vi "RemoteVI Encode Rect PNG.vi"(8 "error in":errorcluster, 9 "compression":i32=1, 10 "rect":cluster{"x":i32, "y":i32, "w":i32, "h":i32}, 11 "pixmap":u32[][](array[numeric])) -> (0 "error out":errorcluster, 3 "png":string)   [LabVIEW 2020, in "RemoteVI.lvlib"]
doc: "Cuts rect out of pixmap (2D U32 [row, column], 0x00RRGGBB) with Array Subset, flattens it to a 24-bit LabVIEW image and encodes it as PNG in memory with LVImageDataToPNGByteArray, the function LabVIEW exports and NI's LV Image to PNG Data.vi calls (Win32\\LabVIEW LVImageDataToPNGByteArray.vi). It is called directly because LabVIEW 2020's LV Image to PNG Data.vi has no compression input and always writes an uncompressed PNG. compression is the zlib level: 0 writes an uncompressed PNG, 1 (default) is the fastest compressing level, 9 the smallest, -1 is zlib's own default (6). It is coerced to -1..9 because the encoder returns an EMPTY png and no error for a level above 9. A rect reaching past the pixmap is clipped by Array Subset. On an error at error in nothing is encoded and png is empty."
uses:
  RemoteVI.lvlib
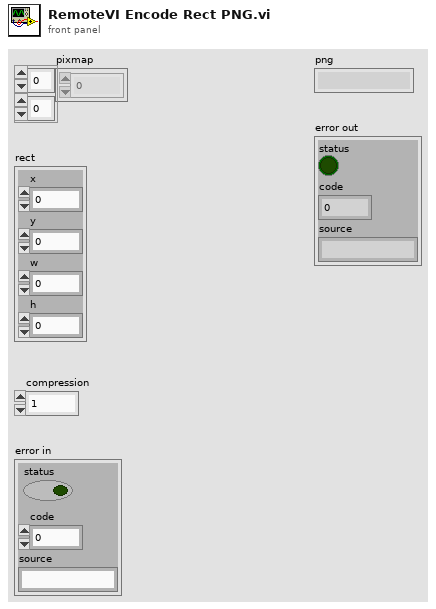
[diagram p1: front panel]
types:
  T1 = typedef "imagedata.ctl" = cluster{"image type":i32, "image depth":i32, "image":u8[], "mask":u8[], "colors":u32[], "Rectangle":cluster{"left":i16, "top":i16, "right":i16, "bottom":i16}}
  T2 = cluster{"left":i16, "top":i16, "right":i16, "bottom":i16}
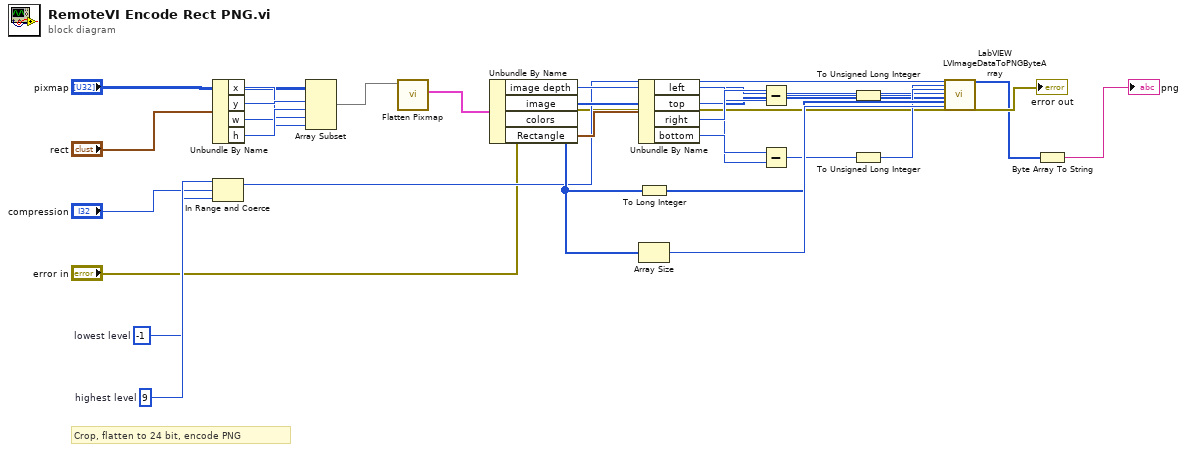
[diagram p0: block diagram]
diagram:
  w6 = 9  # highest level
  w5 = -1  # lowest level
  # "Crop, flatten to 24 bit, encode PNG"
  n1 = Unbundle By Name("rect") -> ("x"=w7:i32, "y"=w8:i32, "w"=w9:i32, "h"=w10:i32)
  n2 = In Range and Coerce(upper limit=w6, x="compression", lower limit=w5) -> (coerced(x)=w11:i32)  [unwired: 1 out]
  n3 = Array Subset(array="pixmap", index (row)=w8, length (row)=w10, index (col)=w7, length (col)=w9) -> (w12:u32[][])
  n4 = call <vilib>:"Flatten Pixmap.vi"("24-bit pixmap"=w12) -> ("image data"=w13:T1)  [unwired: 10 in]
  n5 = Unbundle By Name(w13) -> ("image depth"=w14:i32, "image"=w15:u8[], "colors"=w16:u32[], "Rectangle"=w17:T2)
  n6 = Unbundle By Name(w17) -> ("left"=w18:i16, "top"=w19:i16, "right"=w20:i16, "bottom"=w21:i16)
  n7 = To Long Integer(number=w16) -> (32bit integer=w26:i32[])
  n8 = Array Size(array=w16) -> (size(s)=w27:i32)
  n9 = Subtract(x=w20, y=w18) -> (x-y=w22:i16)
  n10 = Subtract(x=w21, y=w19) -> (x-y=w23:i16)
  n11 = To Unsigned Long Integer(number=w22) -> (unsigned 32bit integer=w24:u32)
  n12 = To Unsigned Long Integer(number=w23) -> (unsigned 32bit integer=w25:u32)
  n13 = call "LabVIEW LVImageDataToPNGByteArray.vi"("compression"=w11, "width"=w24, "height"=w25, "depth"=w14, "imageBuf"=w15, "colorTable"=w26, "colorTableSize"=w27, "error in"="error in") -> ("png data"=w28:u8[], "error out"=→"error out":errorcluster)  [unwired: 18 in]
  n14 = Byte Array To String(unsigned byte array=w28) -> (string=→"png":string)
